vi "Func - VarMan Error handler.vi"(5 "InstanceRef":T2, 6 "error in":bool, 7 "VM error code":T1 items=["No error", "Invalid variable type", "Variable not found", "Variable already exists", "Invalid context handle", "Input error", "Invalid data format", "No history attached", "History already attached", "Invalid history parameters", "Wrong variable name", "Wrong alias name", "Non-unique alias", "Alias not found", "No alias associated", "Alias already associated", "Wrong context name", "Non-unique context name", "Context name not found", "Invalid parameter", "Generic error", "Memory Full", "Unrecognized LV error", "Unknown error code"], 9 "var name":string) -> (0 "error out":bool, 1 "dup VM error code":T1 items=["No error", "Invalid variable type", "Variable not found", "Variable already exists", "Invalid context handle", "Input error", "Invalid data format", "No history attached", "History already attached", "Invalid history parameters", "Wrong variable name", "Wrong alias name", "Non-unique alias", "Alias not found", "No alias associated", "Alias already associated", "Wrong context name", "Non-unique context name", "Context name not found", "Invalid parameter", "Generic error", "Memory Full", "Unrecognized LV error", "Unknown error code"], 3 "dup var name":string)   [LabVIEW 2021]
doc: "This VI handles errors returned by VarMan VIs. Refer to the VI help for more details.\n\n::: CalcExpress Toolkit :::\nCopyright (c) 2000-2026 Konstantin Shifershteyn. All rights reserved."
uses:
  cetypes.llb/VarMan Error Code.ctl
  cetypes.llb/CalcExpress Instance RefNum.ctl
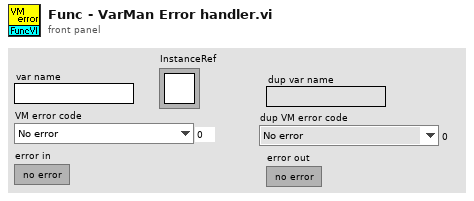
[diagram p1: front panel]
types:
  T1 = typedef "VarMan Error Code.ctl" = u16
  T2 = typedef "CalcExpress Instance RefNum.ctl" = refnum<k1>
  T3 = typedef "VarMan Variable Context Handle.ctl" = i32
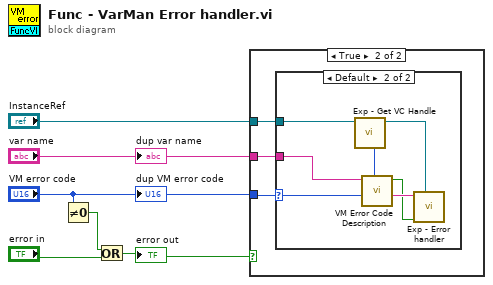
[diagram p0: block diagram]
diagram:
  n1 = Not Equal To 0?(x="VM error code") -> (x != 0?=w6:bool)
  n2 = Or(x=w6, y="error in") -> (x .or. y?=w4:bool)
  "error out" <- w4
  n3 = case shown="True" w4 {
    tunnel: "VM error code" -> [_ w9]
    tunnel: "var name" -> [_ w8]
    tunnel: "InstanceRef" -> [_ w7]
    frame False {
    }
    frame True {
      n4 = case shown="Default" w9 {
        selector: w9 -> [_ w12]
        tunnel: w8 -> [_ w11]
        tunnel: w7 -> [_ w10]
        frame 0, 5 {
        }
        frame Default {
          n5 = call "Exp - Get VC Handle.vi"("InstanceRef"=w10) -> ("dup InstanceRef"=w13:T2, "VC Handle"=w14:T3)  [unwired: 5 in, 2 out]
          n6 = call "VM Error Code Description.vi"("VC Handle"=w14, "VarMan Engine error"=w12, "name spec"=w11) -> ("error description"=w16:string, "error ?"=w15:bool)  [unwired: 6 in, 1 out]
          n7 = call "Exp - Error handler.vi"("InstanceRef"=w13, "error in"=w15, "error message in"=w16) -> ()  [unwired: 6 in, 3 out]
        }
      }
    }
  }
  "dup var name" <- "var name"
  "dup VM error code" <- "VM error code"
